vi "libssh2_scp_recv2.vi"(8 "error in (no error)":errorcluster, 10 "path":string, 11 "session":T3) -> (0 "error out":errorcluster, 2 "stat":T1, 3 "channel":T2)   [LabVIEW 2017, in "libssh2.lvlib"]
doc: "Request a file from an SSH server. When successful, returns a channel instance and the remote file's size, mode, mtime, and atime."
uses:
  libssh2.lvlib
  Session Refnum.ctl
  Channel Refnum.ctl
  libssh2_struct_stat.ctl
  Not A Session.vi
  <vilib>/Utility/error.llb/Error Cluster From Error Code.vi
  Global Settings.vi
  Read Session Refnum.vi
  <vilib>/Utility/semaphor.llb/Acquire Semaphore.vi
  <vilib>/Utility/semaphor.llb/Release Semaphore.vi
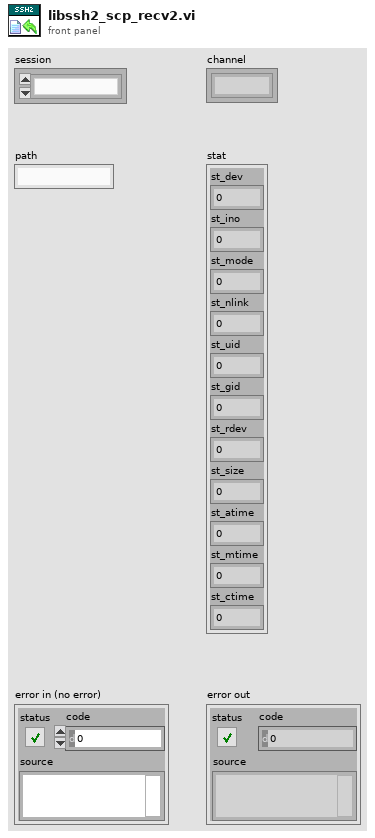
[diagram p1: front panel]
types:
  T1 = typedef "libssh2.lvlib/libssh2_struct_stat.ctl" = cluster{"st_dev":u64, "st_ino":u16, "st_mode":u16, "st_nlink":i16, "st_uid":i16, "st_gid":i16, "st_rdev":u32, "st_size":i64, "st_atime":i64, "st_mtime":i64, "st_ctime":i64}
  T2 = typedef "libssh2.lvlib/Channel Refnum.ctl" = refnum<k1>
  T3 = typedef "libssh2.lvlib/Session Refnum.ctl" = refnum<k1>
  T4 = cluster{"st_dev":u64, "st_ino":u16, "st_mode":u16, "st_nlink":i16, "st_uid":i16, "st_gid":i16, "<padding>":i16, "st_rdev":u32, "st_size":i64, "st_atime":i64, "st_mtime":i64, "st_ctime":i64}
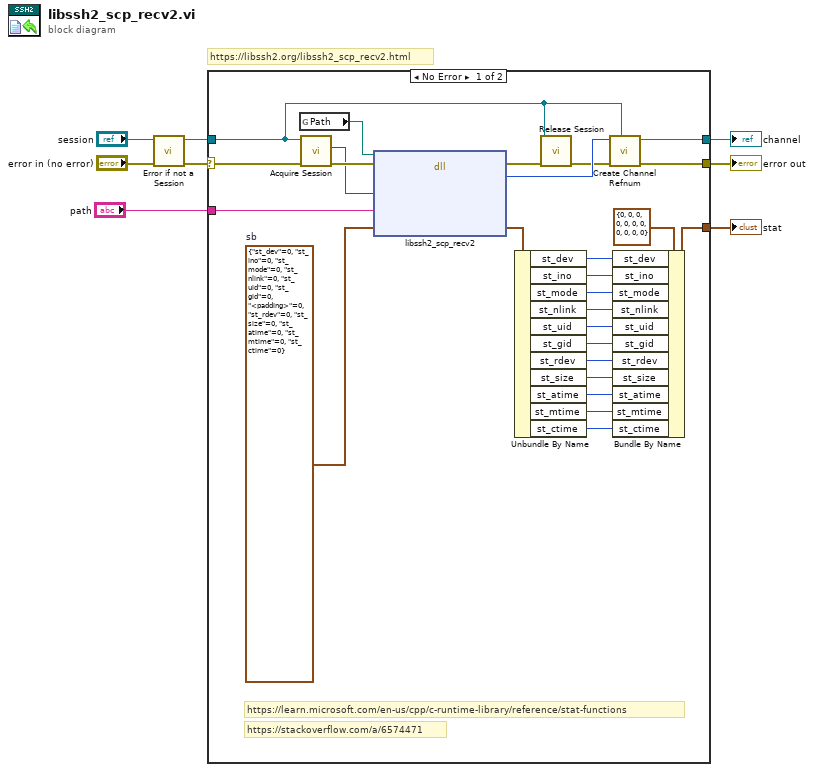
[diagram p0: block diagram]
diagram:
  # "https://libssh2.org/libssh2_scp_recv2.html"
  n1 = call "Error if not a Session.vi"("error in (no error)"="error in (no error)", "session"="session") -> ("error out"=w5:errorcluster, "session out"=w3:T3)  [unwired: 8 in]
  n2 = case shown="No Error" w5 {
    selector: w5 -> [w28 w35]
    tunnel: w3 -> [w9 _]
    tunnel: [w31 w35] -> w8
    tunnel: [w29 _] -> w7
    tunnel: "path" -> [w26 _]
    tunnel: [w11 _] -> w1
    frame No Error {
      w25 = T4 {"st_dev"=0, "st_ino"=0, "st_mode"=0, "st_nlink"=0, "st_uid"=0, "st_gid"=0, "<padding>"=0, "st_rdev"=0, "st_size"=0, "st_atime"=0, "st_mtime"=0, "st_ctime"=0}  # sb
      # "https://stackoverflow.com/a/6574471"
      # "https://learn.microsoft.com/en-us/cpp/c-runtime-library/reference/stat-functions"
      n3 = global read "Global Settings.vi" "Path"() -> (w27:path)
      n4 = call "Acquire Session.vi"("error in (no error)"=w28, "session"=w9) -> ("error out"=w33:errorcluster, "LIBSSH2_SESSION*"=w32:u64)  [unwired: 7 in, 1 out]
      n5 = dll-call lib="?" fn="libssh2_scp_recv2"(path in=w27, error in=w33, "session"=w32, "path"=w26, "sb"=w25) -> (error out=w34:errorcluster, "return value"=w30:u64, "sb"=w24:T4)  [unwired: 3 in, 1 out]
      n6 = Unbundle By Name(w24) -> ("st_dev"=w22:u64, "st_ino"=w21:u16, "st_mode"=w20:u16, "st_nlink"=w19:i16, "st_uid"=w18:i16, "st_gid"=w17:i16, "st_rdev"=w16:u32, "st_size"=w15:i64, "st_atime"=w14:i64, "st_mtime"=w13:i64, "st_ctime"=w12:i64)
      n7 = call "Release Session.vi"("error in (no error)"=w34, "session"=w9) -> ("error out"=w10:errorcluster)  [unwired: 9 in]
      n8 = call "Create Channel Refnum.vi"("session"=w9, "error in (no error)"=w10, "LIBSSH2_CHANNEL*"=w30) -> ("error out"=w31:errorcluster, "channel"=w29:T2)  [unwired: 7 in]
      n9 = Bundle By Name(cluster=T1 {"st_dev"=0, "st_ino"=0, "st_mode"=0, "st_nlink"=0, "st_uid"=0, "st_gid"=0, "st_rdev"=0, "st_size"=0, "st_atime"=0, "st_mtime"=0, "st_ctime"=0} ("sb"), "st_dev"=w22, "st_ino"=w21, "st_mode"=w20, "st_nlink"=w19, "st_uid"=w18, "st_gid"=w17, "st_rdev"=w16, "st_size"=w15, "st_atime"=w14, "st_mtime"=w13, "st_ctime"=w12) -> (w11:T1)
    }
    frame Error {
    }
  }
  "error out" <- w8
  "channel" <- w7
  "stat" <- w1
